vi "Room_Load.vi"(0 "Room ID":string="005", 11 "error in":errorcluster) -> (4 "Tiles":u8[][](array[numeric]), 15 "error out":errorcluster)   [LabVIEW 2020, in "GH_Level.lvlib"]
doc: "Reads Resources\\Levels\\room_<Room ID>.txt into a 2D tile array (row, column), 40 x 20 tiles of 32 px. Tile values: . 0 empty, # 1 wall, = 2 thin floor, ~ 3 vanishing floor, H 4 ladder, | 5 pole, : 6 rope, < 7 and > 8 conveyor, R B Y 10-12 doors, r b y 13-15 keys, g 16 gold coin, G 17 gold hoard, T 18 torch, S 19 spider, Z 20 snake, K 21 skull, P 22 start."
uses:
  GH_Level.lvlib
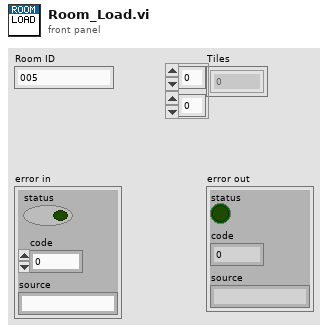
[diagram p1: front panel]
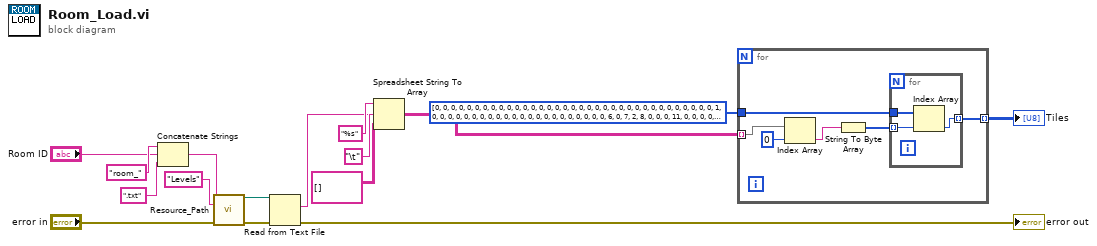
[diagram p0: block diagram]
diagram:
  n1 = Concatenate Strings("room_", "Room ID", ".txt") -> (w5:string)
  n2 = call "Resource_Path.vi"("File name"=w5, "Subfolder"="Levels", "error in"="error in") -> ("Path"=w7:path, "error out"=w8:errorcluster)  [unwired: 11 in]
  n3 = Read from Text File(file (use dialog)=w7, error in=w8) -> (text=w9:string, error out=→"error out":errorcluster)  [unwired: 2 in, 2 out]
  n4 = Spreadsheet String To Array(delimiter (Tab)="\t", format string="%s", spreadsheet string=w9, array type (2D Dbl)=string[][] []) -> (array=w14:string[][])
  n5 = for {
    tunnel: u8[] [0, 0, 0, 0, 0, 0, 0, 0, 0, 0, 0, 0, 0, 0, 0, 0, 0, 0, 0, 0, 0, 0, 0, 0, 0, 0, 0, 0, 0, 0, 0, 0, 0, 0, 0, 1, 0, 0, 0, 0, 0, 0, 0, 0, 0, 0, 0, 0, 0, 0, 0, 0, 0, 0, 0, 0, 0, 0, 6, 0, 7, 2, 8, 0, 0, 0, 11, 0, 0, 0, 0, 17, 4, 0, 0, 21, 0, 0, 0, 0, 22, 0, 10, 19, 18, 0, 0, 0, 0, 12, 20, 0, 0, 0, 0, 0, 0, 0, 14, 0, 0, 0, 0, 16, 0, 0, 0, 0, 0, 0, 0, 0, 0, 0, 13, 0, 0, 0, 0, 0, 0, 15, 0, 0, 5, 0, 3, 0, 0, 0, 0, 0, 0, 0, 0, 0, 0, 0, 0, 0, 0, 0, 0, 0, 0, 0, 0, 0, 0, 0, 0, 0, 0, 0, 0, 0, 0, 0, 0, 0, 0, 0, 0, 0, 0, 0, 0, 0, 0, 0, 0, 0, 0, 0, 0, 0, 0, 0, 0, 0, 0, 0, 0, 0, 0, 0, 0, 0, 0, 0, 0, 0, 0, 0, 0, 0, 0, 0, 0, 0, 0, 0, 0, 0, 0, 0, 0, 0, 0, 0, 0, 0, 0, 0, 0, 0, 0, 0, 0, 0, 0, 0, 0, 0, 0, 0, 0, 0, 0, 0, 0, 0, 0, 0, 0, 0, 0, 0, 0, 0, 0, 0, 0, 0, 0, 0, 0, 0, 0, 0, 0, 0, 0, 0, 0, 0] ("Tile value per character") -> [w18]
    tunnel: w14 -> [w17] mode=indexing
    tunnel: [w22] -> w16 mode=indexing
    n6 = Index Array(array=w17, index=0) -> (element=w20:string)
    n7 = String To Byte Array(string=w20) -> (unsigned byte array=w21:u8[])
    n8 = for {
      tunnel: w18 -> [w24]
      tunnel: w21 -> [w23] mode=indexing
      tunnel: [w25] -> w22 mode=indexing
      n9 = Index Array(array=w24, index=w23) -> (element=w25:u8)
    }
  }
  "Tiles" <- w16
